vi "error handling.vi"(8 "error in (no error)":errorcluster, 11 "return val":i32) -> (0 "error out":errorcluster)   [LabVIEW 2023, in "xnet_canopen.lvlib"]
uses:
  xnet_canopen.lvlib
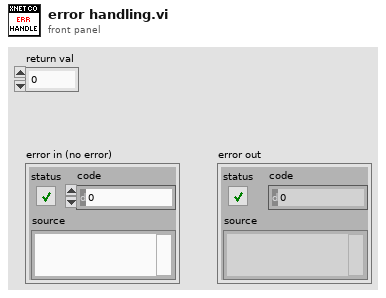
[diagram p1: front panel]
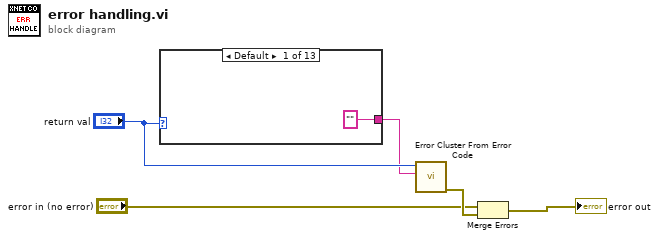
[diagram p0: block diagram]
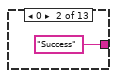
[diagram p2: hidden frame]
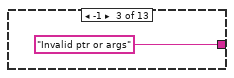
[diagram p3: hidden frame]
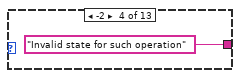
[diagram p4: hidden frame]
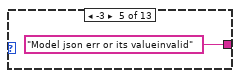
[diagram p5: hidden frame]
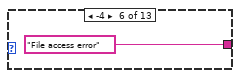
[diagram p6: hidden frame]
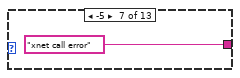
[diagram p7: hidden frame]
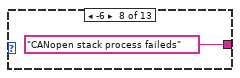
[diagram p8: hidden frame]
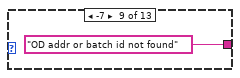
[diagram p9: hidden frame]
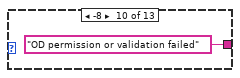
[diagram p10: hidden frame]
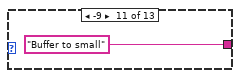
[diagram p11: hidden frame]
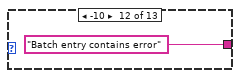
[diagram p12: hidden frame]
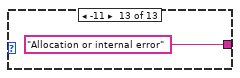
[diagram p13: hidden frame]
diagram:
  n1 = case shown="Default" "return val" {
    tunnel: ["" "Success" "Invalid ptr or args" "Invalid state for such operation" "Model json err or its valueinvalid" "File access error" "xnet call error" "CANopen stack process faileds" "OD addr or batch id not found" "OD permission or validation failed" "Buffer to small" "Batch entry contains error" "Allocation or internal error"] -> w4
    frame Default {
    }
    frame 0 {
    }
    frame -1 {
    }
    frame -2 {
    }
    frame -3 {
    }
    frame -4 {
    }
    frame -5 {
    }
    frame -6 {
    }
    frame -7 {
    }
    frame -8 {
    }
    frame -9 {
    }
    frame -10 {
    }
    frame -11 {
    }
  }
  n2 = call <vilib>:"Error Cluster From Error Code.vi"("error message (\"\")"=w4, "error code (0)"="return val") -> ("error out"=w3:errorcluster)  [unwired: 7 in]
  n3 = Merge Errors("error in (no error)", w3) -> (→"error out":errorcluster)
